vi "Acquire.vi"(8 "error in (no error)":errorcluster, 11 "Measurement in":refnum<class "Measurement.lvclass">) -> (0 "error out":errorcluster, 3 "Measurement out":refnum<class "Measurement.lvclass">)   [LabVIEW 2017, in "Measurement Actor.lvlib" / "Measurement.lvclass"]
uses:
  Measurement.lvclass
  C:/Program Files (x86)/National Instruments/LabVIEW 2017/vi.lib/ActorFramework/Actor/Actor.lvclass
  Measurement.lvclass/Measurement.ctl
  Configuration/Step Configuration.lvclass/Step Configuration.ctl
  Logger/config/Logger Configuration.lvclass/Logger Configuration.ctl
  <vilib>/ActorFramework/Actor/Actor.lvclass/Actor.ctl
  <vilib>/ActorFramework/Message Enqueuer/Message Enqueuer.lvclass/Message Enqueuer.ctl
  Configuration/Accessors/Read Logger Config.vi
  Logger/config/Read Logging Settings.vi
  <vilib>/ActorFramework/Message Enqueuer/Init from Existing Queue.vi
  <vilib>/ActorFramework/Message Enqueuer/Enqueue.vi
  Measurement Messages/Update CVT Msg/Update CVT Msg.lvclass
  C:/Program Files (x86)/National Instruments/LabVIEW 2017/vi.lib/ActorFramework/Message/Message.lvclass
  Measurement Messages/Publish Latest Data to Logger Msg/Publish Latest Data to Logger Msg.lvclass
  Messages/Measure Msg/Measure Msg.lvclass
  Messages/Acquire Msg/Acquire Msg.lvclass
  <vilib>/ActorFramework/Message Priority Queue/Priority Enqueue.vi
  Configuration/Step Configuration.lvclass
  <vilib>/ActorFramework/Message Enqueuer/Message Enqueuer.lvclass
  Logger/config/Logger Configuration.lvclass
  <vilib>/ActorFramework/Actor/Actor.lvclass
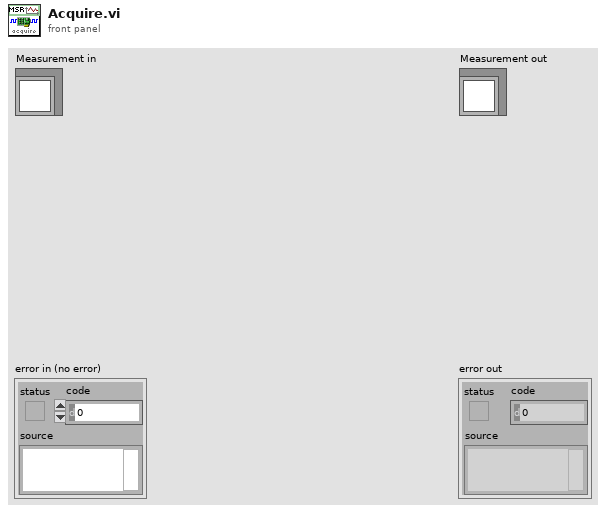
[diagram p1: front panel]
types:
  T1 = typedef "Measurement Actor.lvlib/Measurement.lvclass/Iteration count.ctl" = cluster{"Desired Iterations":i32, "Current":i32}
  T2 = cluster{"File Name":string, "Upload Files to SystemLink Server":bool, "Max Samples Per File":i32, "Folder Location":path, "Logging":bool}
  T3 = cluster{"Run indefinitely":bool, "Iterations":i32}
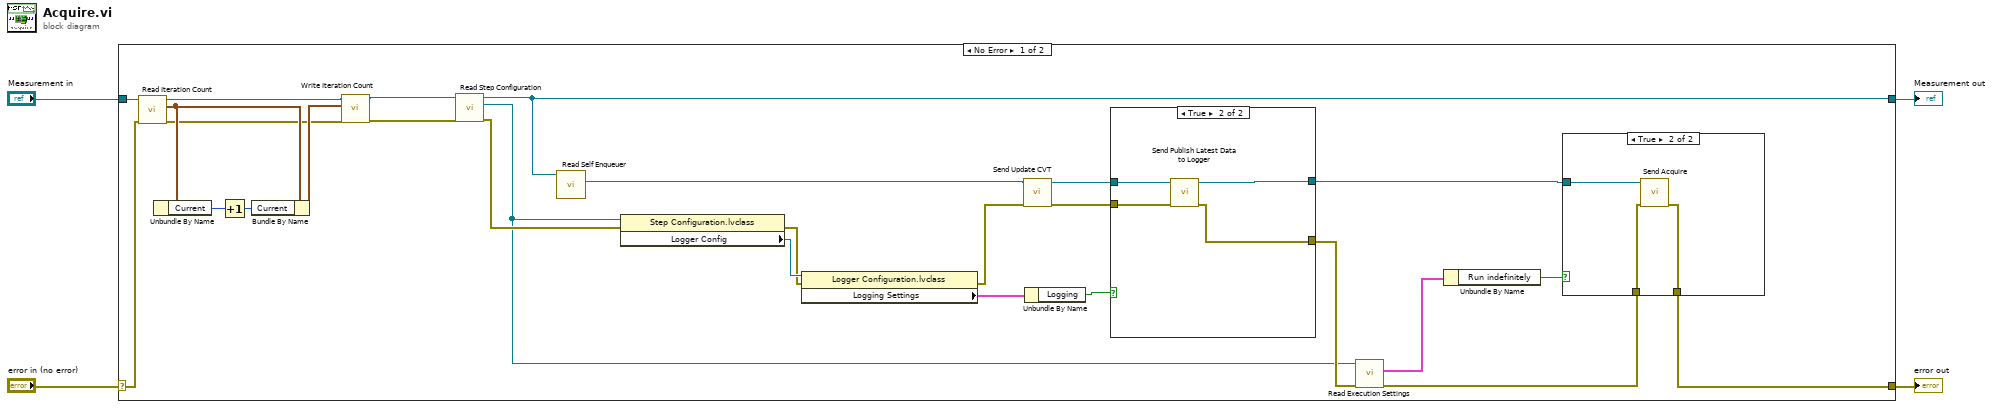
[diagram p0: block diagram]
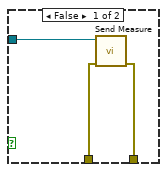
[diagram p3: hidden frame]
diagram:
  n1 = case shown="No Error" "error in (no error)" {
    selector: "error in (no error)" -> [w19 w45]
    tunnel: [w8 w45] -> w3
    tunnel: [w22 w44] -> w1
    tunnel: "Measurement in" -> [w28 w44]
    frame No Error {
      n2 = call "Read Iteration Count.vi"("error in (no error)"=w19, "Measurement in"=w28) -> ("error out"=w21:errorcluster, "Iteration Count"=w29:T1, "Measurement out"=w26:refnum<class "Measurement.lvclass">)  [unwired: 7 in]
      n3 = Unbundle By Name(w29) -> ("Current"=w31:i32)
      n4 = Increment(x=w31) -> (x+1=w30:i32)
      n5 = Bundle By Name(cluster=w29, "Current"=w30) -> (w27:T1)
      n6 = call "Write Iteration Count.vi"("error in (no error)"=w21, "Iteration Count"=w27, "Measurement in"=w26) -> ("error out"=w20:errorcluster, "Measurement out"=w25:refnum<class "Measurement.lvclass">)  [unwired: 7 in]
      n7 = call "Read Step Configuration.vi"("error in (no error)"=w20, "Measurement in"=w25) -> ("error out"=w18:errorcluster, "Measurement Actor.lvlib:Step Configuration.lvclass"=w10:refnum<class "Step Configuration.lvclass">, "Measurement out"=w22:refnum<class "Measurement.lvclass">)  [unwired: 7 in]
      n8 = call <vilib>:"Read Self Enqueuer.vi"("Actor"=w22) -> ("Self Enqueuer"=w6:refnum<class "Message Enqueuer.lvclass">)  [unwired: 10 in]
      n9 = property class="Step Configuration.lvclass"(reference=w10, error in=w18) -> (error out=w15:errorcluster, "Logger Config"=w17:refnum<class "Logger Configuration.lvclass">)  [unwired: 1 out]
      n10 = property class="Logger Configuration.lvclass"(reference=w17, error in=w15) -> (error out=w13:errorcluster, "Logging Settings"=w16:T2)  [unwired: 1 out]
      n11 = call "Send Update CVT.vi"("error in (no error)"=w13, "Message Enqueuer"=w6) -> ("error out"=w7:errorcluster, "Message Enqueuer out"=w5:refnum<class "Message Enqueuer.lvclass">)  [unwired: 8 in]
      n12 = Unbundle By Name(w16) -> ("Logging"=w14:bool)
      n13 = case shown="True" w14 {
        tunnel: w5 -> [w33 w37]
        tunnel: [w33 w36] -> w11
        tunnel: w7 -> [w32 w35]
        tunnel: [w32 w34] -> w12
        frame False {
        }
        frame True {
          n14 = call "Send Publish Latest Data to Logger.vi"("error in (no error)"=w35, "Message Enqueuer"=w37) -> ("error out"=w34:errorcluster, "Message Enqueuer out"=w36:refnum<class "Message Enqueuer.lvclass">)  [unwired: 8 in]
        }
      }
      n15 = call "Read Execution Settings.vi"("error in (no error)"=w12, "Step Configuration in"=w10) -> ("error out"=w9:errorcluster, "Execution Settings"=w24:T3)  [unwired: 7 in, 1 out]
      n16 = Unbundle By Name(w24) -> ("Run indefinitely"=w23:bool)
      n17 = case shown="True" w23 {
        tunnel: w11 -> [w40 w43]
        tunnel: w9 -> [w39 w42]
        tunnel: [w38 w41] -> w8
        frame False {
          n18 = call "Send Measure.vi"("error in (no error)"=w39, "Message Enqueuer in"=w40) -> ("error out"=w38:errorcluster)  [unwired: 8 in, 1 out]
        }
        frame True {
          n19 = call "Send Acquire.vi"("error in (no error)"=w42, "Message Enqueuer in"=w43) -> ("error out"=w41:errorcluster)  [unwired: 8 in, 1 out]
        }
      }
    }
    frame Error {
    }
  }
  "error out" <- w3
  "Measurement out" <- w1
